vi "Handle Template.vi"(7 "Processing In":refnum<class "Processing.lvclass">, 8 "error in (no error)":errorcluster, 10 "Path":path, 11 "TemplatedFileServe in":refnum<class "TemplatedFileServe.lvclass">) -> (0 "error out":errorcluster, 2 "Response":refnum<class "Response.lvclass">, 3 "TemplatedFileServe out":refnum<class "TemplatedFileServe.lvclass">, 5 "Processing":refnum<class "Processing.lvclass">)   [LabVIEW 2020, in "HTTP Server.lvlib" / "TemplatedFileServe.lvclass"]
uses:
  TemplatedFileServe.lvclass
  lv-http-util/HTTP Utils/Response/Response.lvclass
  Processing/Processing.lvclass
  TemplateService/TemplateService.lvclass
  C:/dev/lv20CE/relink/lv-http-server/HTTP Server/Service/Service.lvclass
  Processing/Processing.lvclass/Processing.ctl
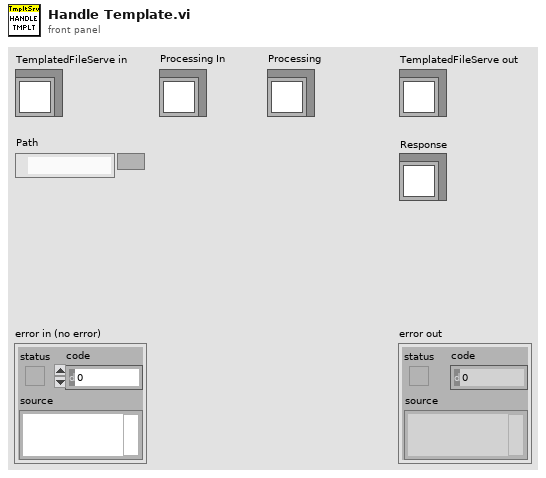
[diagram p1: front panel]
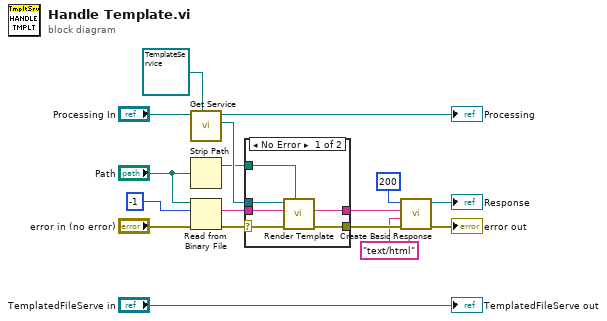
[diagram p0: block diagram]
diagram:
  n1 = call "Get Service.vi"("Service Type"=refnum<class "TemplateService.lvclass"> refnum ("HTTP Server:TemplateService.lvclass"), "Processing in"="Processing In") -> ("Service"=w13:refnum<class "TemplateService.lvclass">, "Processing out"=→"Processing":refnum<class "Processing.lvclass">)  [unwired: 7 in, 1 out]
  n2 = Strip Path(path="Path") -> (stripped path=w1:path)  [unwired: 1 out]
  n3 = Read from Binary File(8:"error in (no error)", 10:-1 ("count (1)"), 11:"Path") -> (0:w10:errorcluster, 2:w11:string)  [unwired: 3 in, 2 out]
  n4 = case shown="No Error" w10 {
    selector: w10 -> [w21 w24]
    tunnel: w13 -> [w23 _]
    tunnel: w11 -> [w22 _]
    tunnel: [w19 w24] -> w17
    tunnel: [w20 _] -> w8
    tunnel: w1 -> [w18 _]
    frame No Error {
      n5 = call-dynamic "Render Template.vi"("Folder"=w18, "error in (no error)"=w21, "Template"=w22, "TemplateService in"=w23) -> ("error out"=w19:errorcluster, "Output"=w20:string)  [unwired: 5 in, 1 out]
    }
    frame Error {
    }
  }
  n6 = call "Create Basic Response.vi"("error in (no error)"=w17, "Content-Type (text/plain)"="text/html", "Payload"=w8, "Status Code"=u16 200) -> ("error out"=→"error out":errorcluster, "Response out"=→"Response":refnum<class "Response.lvclass">)  [unwired: 6 in]
  "TemplatedFileServe out" <- "TemplatedFileServe in"
